vi "Begin Step.vi"(8 "error in":errorcluster, 11 "Sequence Executor in":refnum<class "Sequence Executor.lvclass">) -> (0 "error out":errorcluster, 3 "Sequence Executor out":refnum<class "Sequence Executor.lvclass">)   [LabVIEW 2026, in "Sequence Executor.lvclass"]
doc: "Helper. Begins step Step Index: its result becomes RUNNING, Phase Settling, Step Start ms -1 (latched by Process Feedback on the next plant sample), Dwell Start ms 0; sends Set Setpoints Msg with the step's three setpoints to the plant and refreshes the displays."
uses:
  Sequence Executor.lvclass
  Sequence Executor.lvclass/Sequence Executor.ctl
  C:/Program Files/National Instruments/LabVIEW 2026/vi.lib/ActorFramework/Actor/Actor.lvclass
  C:/Users/DynaAdmin/PycharmProjects/Universal-sequence-executor-AF/src/Executor/Sequence Executor.lvclass
  <vilib>/ActorFramework/Message Enqueuer/Message Enqueuer.lvclass
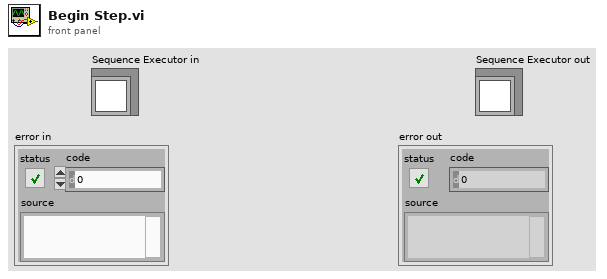
[diagram p1: front panel]
types:
  T1 = cluster{"pressure_sp_bar":dbl, "flow_sp_lpm":dbl, "displacement_sp_mm":dbl}
  T2 = typedef "Sequence File.ctl" = cluster{"sequence_id":string, "description":string, "total_steps":i32, "steps":T3[]}
  T3 = typedef "Step Config.ctl" = cluster{"step_no":i32, "step_name":string, "command_type":string, "pressure_sp_bar":dbl, "flow_sp_lpm":dbl, "displacement_sp_mm":dbl, "monitored_io":string, "tolerance_bar":dbl, "dwell_time_ms":i32, "timeout_ms":i32, "expected_result":string}
  T4 = typedef "Step Result.ctl" = cluster{"step_no":i32, "step_name":string, "result":string, "reason":string, "measured":dbl, "target":dbl, "duration_ms":dbl}
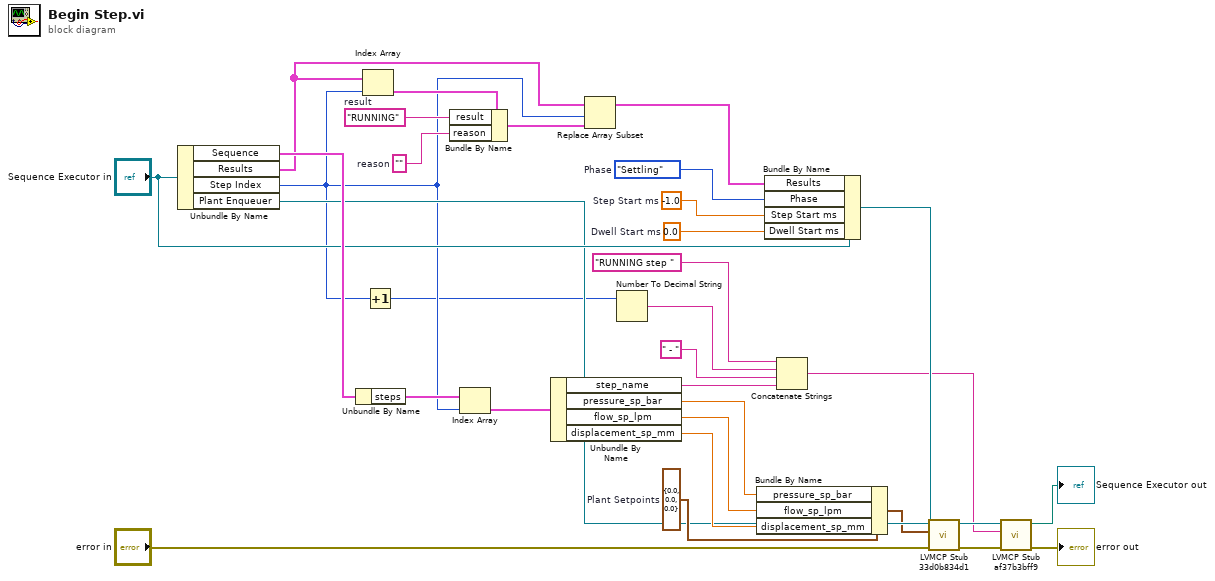
[diagram p0: block diagram]
diagram:
  w16 = 0.0  # Dwell Start ms
  w17 = -1.0  # Step Start ms
  w18 = enum16{"Idle", "Settling", "Dwell", "Complete"}."Settling"  # Phase
  w23 = ""  # reason
  w24 = "RUNNING"  # result
  w25 = T1 {"pressure_sp_bar"=0.0, "flow_sp_lpm"=0.0, "displacement_sp_mm"=0.0}  # Plant Setpoints
  n1 = Unbundle By Name("Sequence Executor in") -> ("Sequence"=w31:T2, "Results"=w21:T4[], "Step Index"=w11:i32, "Plant Enqueuer"=w14:refnum<class "Message Enqueuer.lvclass">)
  n2 = Unbundle By Name(w31) -> ("steps"=w30:T3[])
  n3 = Index Array(array=w21, index=w11) -> (element=w22:T4)
  n4 = Increment(x=w11) -> (x+1=w10:i32)
  n5 = Bundle By Name(cluster=w22, "result"=w24, "reason"=w23) -> (w20:T4)
  n6 = Index Array(array=w30, index=w11) -> (element=w29:T3)
  n7 = Unbundle By Name(w29) -> ("step_name"=w6:string, "pressure_sp_bar"=w28:dbl, "flow_sp_lpm"=w27:dbl, "displacement_sp_mm"=w26:dbl)
  n8 = Replace Array Subset(array=w21, new element=w20, index=w11) -> (w19:T4[])
  n9 = Number To Decimal String(number=w10) -> (decimal integer string=w8:string)  [unwired: 1 in]
  n10 = Bundle By Name(cluster=w25, "pressure_sp_bar"=w28, "flow_sp_lpm"=w27, "displacement_sp_mm"=w26) -> (w13:T1)
  n11 = Bundle By Name(cluster="Sequence Executor in", "Results"=w19, "Phase"=w18, "Step Start ms"=w17, "Dwell Start ms"=w16) -> (w5:refnum<class "Sequence Executor.lvclass">)
  n12 = Concatenate Strings("RUNNING step ", w8, " - ", w6) -> (w4:string)
  n13 = call <userlib>:"LVMCP Stub 33d0b834d1.vi"("error in (no error)"="error in", "Plant Setpoints"=w13, "Message Enqueuer"=w14) -> ("error out"=w3:errorcluster)  [unwired: 7 in, 1 out]
  n14 = call <userlib>:"LVMCP Stub af37b3bff9.vi"("error in"=w3, "Status"=w4, "Sequence Executor in"=w5) -> ("error out"=→"error out":errorcluster, "Sequence Executor out"=→"Sequence Executor out":path)  [unwired: 7 in]
